vi "Convert Press. Regul. Set Bar to Voltage.vi"(11 "Set pressure Hybrid Heart (Bar)":dbl) -> (3 "Numeric":dbl)   [LabVIEW 2024]
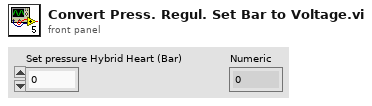
[diagram p1: front panel]
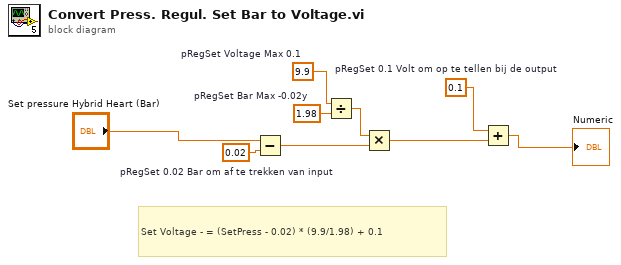
[diagram p0: block diagram]
diagram:
  w6 = 0.1  # pRegSet 0.1 Volt om op te tellen bij de output
  w3 = 1.98  # pRegSet Bar Max -0.02y
  w9 = 9.9  # pRegSet Voltage Max 0.1
  w1 = 0.02  # pRegSet 0.02 Bar om af te trekken van input
  # "Set Voltage - = (SetPress - 0.02) * (9.9/1.98) + 0.1"
  n1 = Subtract(x="Set pressure Hybrid Heart (Bar)", y=w1) -> (x-y=w2:dbl)
  n2 = Divide(x=w9, y=w3) -> (x/y=w4:dbl)
  n3 = Multiply(x=w4, y=w2) -> (x*y=w5:dbl)
  n4 = Add(x=w6, y=w5) -> (x+y=→"Numeric":dbl)
